vi "GIHM_Charge Popup.vi"(2 "error in (no error)":errorcluster, 3 "Message":T2="Action réalisée en fonction du problème observé", 4 "Problème observé :":T3="Problème observé sur nom régulateur\r") -> (0 "error out":errorcluster)   [LabVIEW 2022 SP3]
doc: "Charge les écrans Popup en les décalant vers le bas puis vers la droite. Quand l'écran est plein, on recommence en haut et à gauche"
uses:
  Enum/Enum r11.ctl
  Enum/Enum r12.ctl
  Enum/Enum r10.ctl
  Variables globales/Variables glob EUROTHERM.vi
panel:
  in  "Type problème":T1
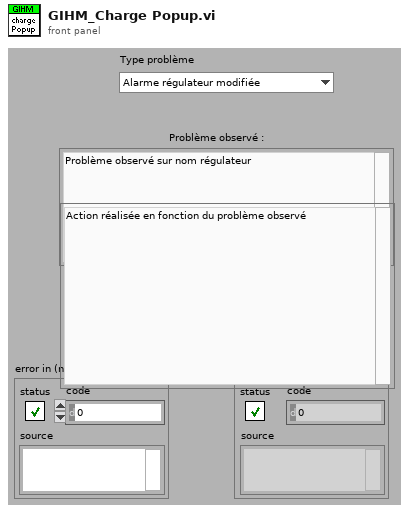
[diagram p1: front panel]
types:
  T1 = typedef "Enum r10.ctl" = enum16{"Alarme régulateur modifiée", "Problème dialogue régulateur"}
  T2 = typedef "Enum r12.ctl" = string
  T3 = typedef "Enum r11.ctl" = string
  T4 = enum32{"Invalid", "Standard", "Closed", "Hidden", "Minimized", "Maximized"}
  T5 = typedef "LVRectTypeDef.ctl" = cluster{"Left":i16, "Top":i16, "Right":i16, "Bottom":i16}
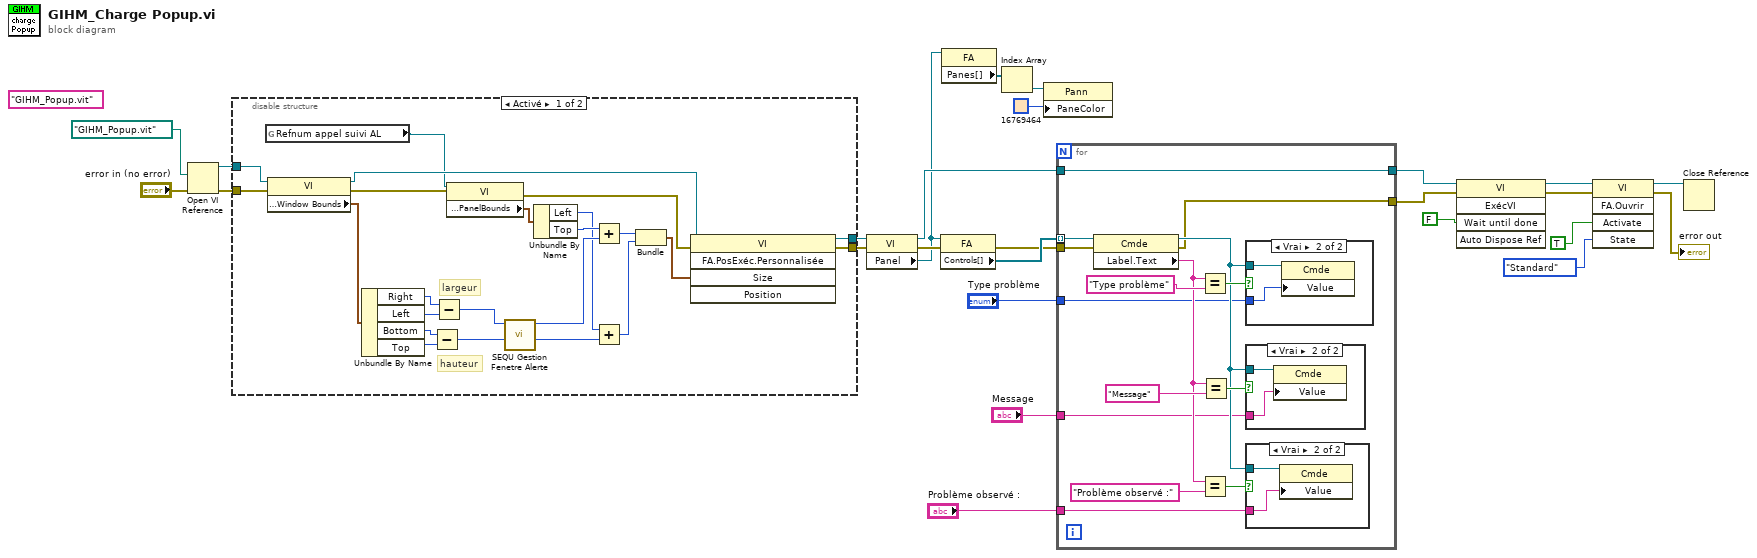
[diagram p0: block diagram]
diagram:
  (unwired) "GIHM_Popup.vit" ("nom ou chemin relatif")
  n1 = Open VI Reference(vi path=path "GIHM_Popup.vit", error in (no error)="error in (no error)") -> (vi reference=w4:refnum<vi>, error out=w2:errorcluster)  [unwired: 1 in, 3 out]
  n2 = disable-structure shown="Activé" {
    disable-tunnel: w4 -> [w31 w51]
    disable-tunnel: [w30 w51] -> w3
    disable-tunnel: w2 -> [w29 w50]
    disable-tunnel: [w28 w50] -> w1
    frame Enabled {
      # "largeur"
      # "hauteur"
      n3 = global read "Variables glob EUROTHERM.vi" "Refnum appel suivi AL"() -> (w27:refnum<vi>)
      n4 = property class="VI"(reference=w31, error in=w29) -> (reference out=w43:refnum<vi>, error out=w44:errorcluster, "Front Panel Window:Window Bounds"=w38:T5)
      n5 = Unbundle By Name(w38) -> ("Right"=w35:i16, "Left"=w34:i16, "Bottom"=w37:i16, "Top"=w36:i16)
      n6 = Subtract(x=w37, y=w36) -> (x-y=w47:i16)
      n7 = Subtract(x=w35, y=w34) -> (x-y=w46:i16)
      n8 = property class="VI"(reference=w27, error in=w44) -> (error out=w45:errorcluster, "Front Panel.PanelBounds"=w42:T5)  [unwired: 1 out]
      n9 = call "SEQU Gestion Fenetre Alerte.vi"("Hauteur"=w47, "Largeur"=w46) -> ("Left"=w48:i32, "Top"=w49:i32)  [unwired: 8 in]
      n10 = Unbundle By Name(w42) -> ("Left"=w33:i16, "Top"=w40:i16)
      n11 = Add(x=w40, y=w49) -> (x+y=w39:i32)
      n12 = Add(x=w33, y=w48) -> (x+y=w32:i32)
      n13 = Bundle(w39, w32) -> (w41:cluster{i32, i32})  [unwired: 1 in]
      n14 = invoke class="VI" method="FA.PosExéc.Personnalisée"(reference=w43, error in=w45, "Size"=w41) -> (reference out=w30:refnum<vi>, error out=w28:errorcluster)  [unwired: 2 in, 3 out]
    }
    frame Disabled {
    }
  }
  n15 = property class="VI"(reference=w3, error in=w1) -> (reference out=w21:refnum<vi>, error out=w23:errorcluster, "Panel"=w13:refnum<vi>)
  n16 = property class="FA"(reference=w13, error in=w23) -> (error out=w8:errorcluster, "Controls[]"=w20:refnum<vi>[])  [unwired: 1 out]
  n17 = property class="FA"(reference=w13) -> ("Panes[]"=w11:refnum<vi>[])  [unwired: 1 in, 2 out]
  n18 = Index Array(array=w11) -> (element=w10:refnum<vi>)  [unwired: 1 in]
  n19 = property class="Pann"(reference=w10, "PaneColor"=u32 16769464) -> ()  [unwired: 1 in, 2 out]
  n20 = for {
    tunnel: [w66] -> w18
    tunnel: w21 -> [w66]
    tunnel: [w53] -> w19
    tunnel: w20 -> [w65] mode=indexing
    tunnel: "Message" -> [w56]
    tunnel: "Type problème" -> [w55]
    tunnel: w8 -> [w54]
    tunnel: "Problème observé :" -> [w52]
    n21 = property class="Cmde"(reference=w65, error in=w54) -> (reference out=w58:refnum<vi>, error out=w53:errorcluster, "Label.Text"=w57:string)
    n22 = Equal?(x=w57, y="Type problème") -> (x = y?=w64:bool)
    n23 = Equal?(x=w57, y="Problème observé :") -> (x = y?=w59:bool)
    n24 = Equal?(x=w57, y="Message") -> (x = y?=w61:bool)
    n25 = case shown="Vrai" w64 {
      tunnel: w58 -> [_ w70]
      tunnel: w55 -> [_ w69]
      frame False {
      }
      frame True {
        n26 = property class="Cmde"(reference=w70, "Value"=w69) -> ()  [unwired: 1 in, 2 out]
      }
    }
    n27 = case shown="Vrai" w61 {
      tunnel: w58 -> [_ w72]
      tunnel: w56 -> [_ w71]
      frame False {
      }
      frame True {
        n28 = property class="Cmde"(reference=w72, "Value"=w71) -> ()  [unwired: 1 in, 2 out]
      }
    }
    n29 = case shown="Vrai" w59 {
      tunnel: w58 -> [_ w68]
      tunnel: w52 -> [_ w67]
      frame False {
      }
      frame True {
        n30 = property class="Cmde"(reference=w68, "Value"=w67) -> ()  [unwired: 1 in, 2 out]
      }
    }
  }
  n31 = invoke class="VI" method="ExécVI"(reference=w18, error in=w19, "Wait until done"=FALSE) -> (reference out=w16:refnum<vi>, error out=w15:errorcluster)  [unwired: 2 in, 3 out]
  n32 = invoke class="VI" method="FA.Ouvrir"(reference=w16, error in=w15, "Activate"=TRUE ("Activer"), "State"=T4."Standard" ("État")) -> (reference out=w9:refnum<vi>, error out=→"error out":errorcluster)  [unwired: 1 in, 3 out]
  n33 = Close Reference(reference=w9) -> ()  [unwired: 1 in, 1 out]
